vi "WLAN_SuperposedFrameBuild_MOD.vi"(4 "Modulation parameter LP":T1, 7 "Alpha":dbl min=0.0 max=1.0 step=0.05 format="%#_13g", 8 "error in (no error)":errorcluster, 9 "data in 2":i8[](array[numeric]) caption="input bit stream", 10 "Modulation parameter HP":T1, 11 "data in":i8[](array[numeric]) caption="input bit stream") -> (0 "error out":errorcluster, 2 "symbolsLP":cdb[](array[numeric]), 3 "symbolsHP":cdb[](array[numeric]))   [LabVIEW 2022 SP3]
panel:
  out "scrambled bits":i8[](array[numeric])
  out "size(s) 5":i32
  out "symbols":cdb[](array[numeric])
  out "output bit stream 4":i8[](array[numeric])
  out "output bit stream 3":i8[](array[numeric])
  out "subarray 2":i8[](array[numeric])
  out "subarray":i8[](array[numeric])
  out "size(s) 2":i32
  out "size(s) 6":i32
  out "size(s) 4":i32
  out "size(s) 3":i32
  out "size(s)":i32
  in  "data in 3":i8[](array[numeric]) caption="input bit stream"
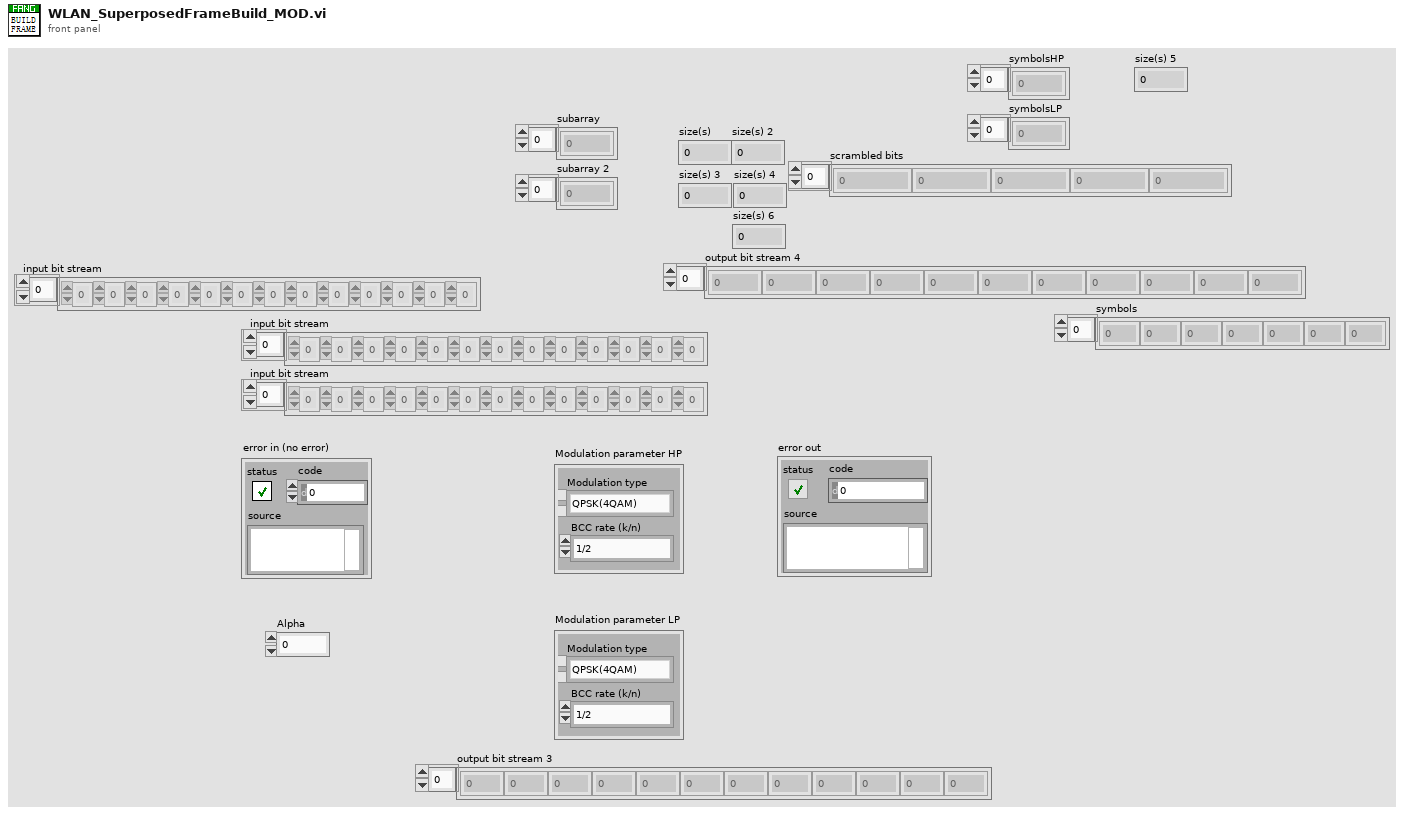
[diagram p1: front panel]
types:
  T1 = cluster{"Modulation type":enum16{"QPSK(4QAM)", "64QAM", "16QAM", "BPSK"}, "BCC rate (k/n)":enum16{"1/2", "2/3", "3/4"}}
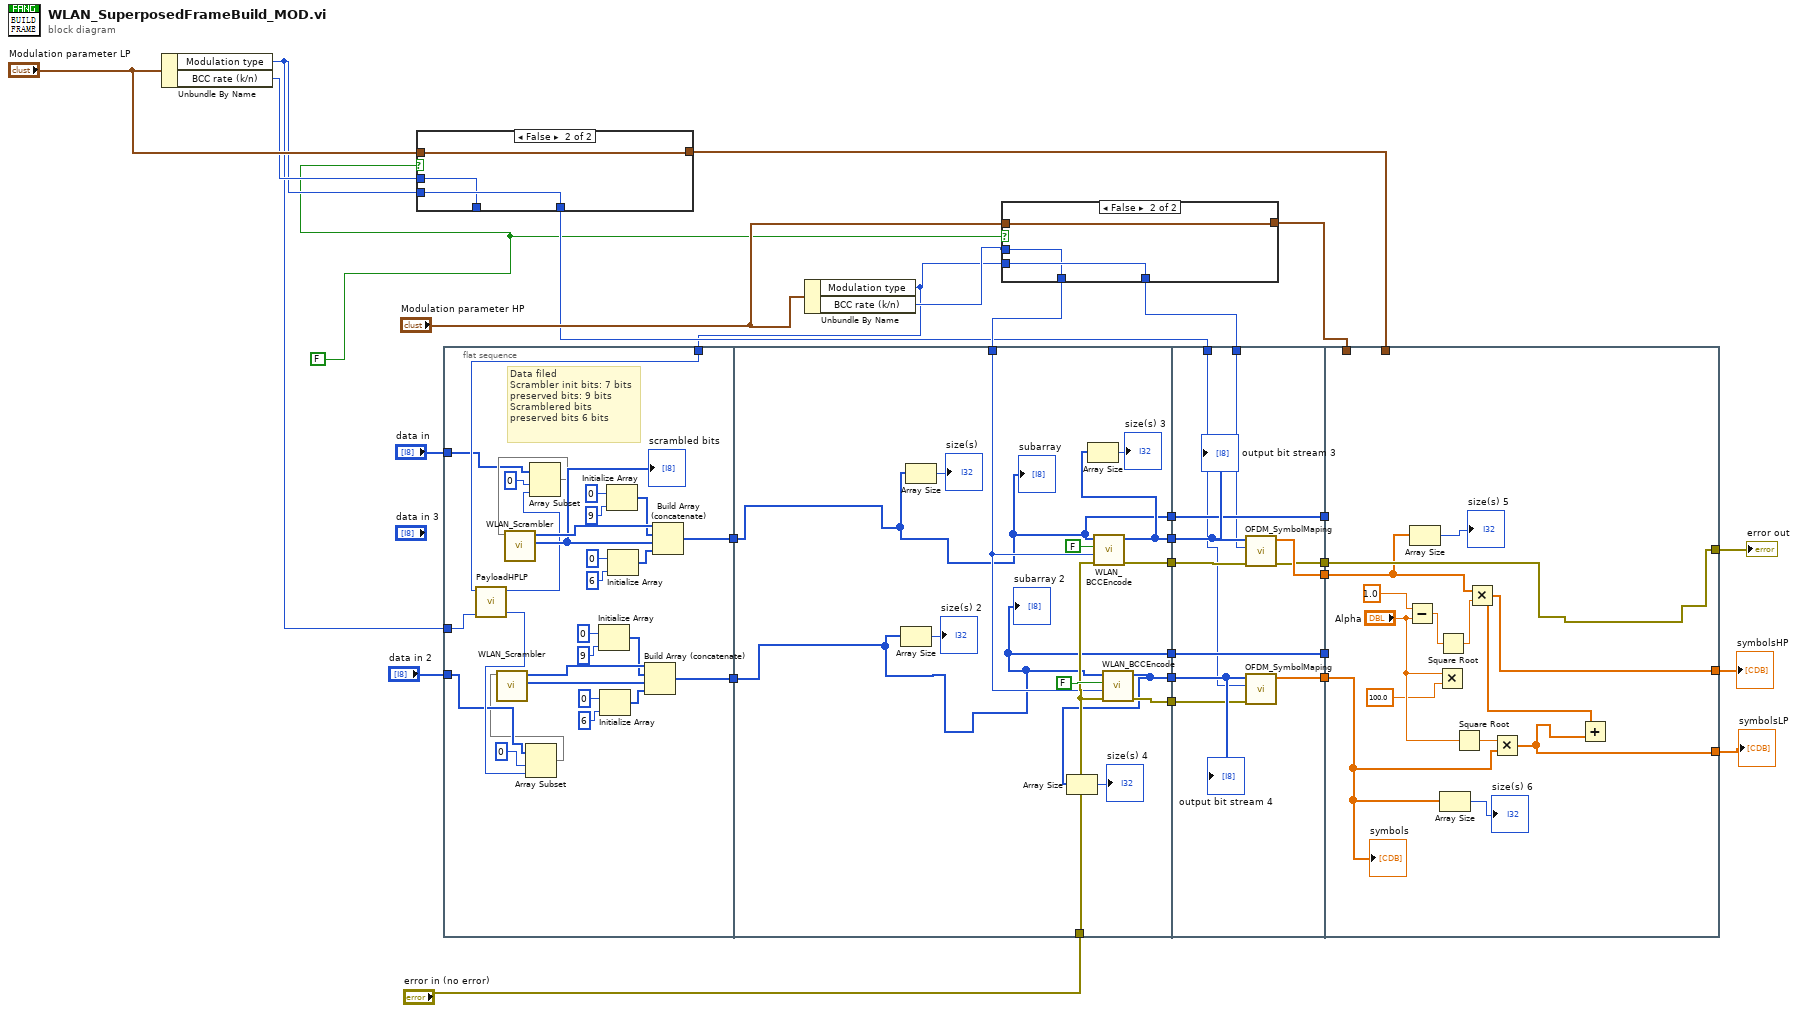
[diagram p0: block diagram]
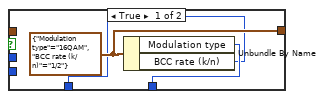
[diagram p2: hidden frame]
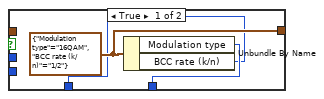
[diagram p3: hidden frame]
diagram:
  w1 = FALSE
  n1 = Unbundle By Name("Modulation parameter LP") -> ("Modulation type"=w5:enum16{"QPSK(4QAM)", "64QAM", "16QAM", "BPSK"}, "BCC rate (k/n)"=w8:enum16{"1/2", "2/3", "3/4"})
  n2 = case shown="False" w1 {
    tunnel: w5 -> [_ w37]
    tunnel: [w34 w37] -> w7
    tunnel: [w33 w36] -> w6
    tunnel: "Modulation parameter LP" -> [_ w36]
    tunnel: [w32 w35] -> _
    tunnel: w8 -> [_ w35]
    frame True {
      w33 = T1 {"Modulation type"=enum."16QAM", "BCC rate (k/n)"=enum."1/2"} ("Modulation parameter")
      n3 = Unbundle By Name(w33) -> ("Modulation type"=w34:enum16{"QPSK(4QAM)", "64QAM", "16QAM", "BPSK"}, "BCC rate (k/n)"=w32:enum16{"1/2", "2/3", "3/4"})
    }
    frame False {
    }
  }
  n4 = flat-sequence {
    tunnel: "data in" -> [w40]
    tunnel: [w57] -> w30
    tunnel: "data in 2" -> [w39]
    tunnel: [w48] -> w20
    tunnel: w5 -> [w47]
    tunnel: w4 -> [w46]
    tunnel: w30 -> [w67]
    tunnel: "error in (no error)" -> [w76]
    tunnel: [w78] -> w28
    tunnel: [w70] -> w27
    tunnel: w11 -> [w75]
    tunnel: [w67] -> w23
    tunnel: w20 -> [w66]
    tunnel: [w66] -> w19
    tunnel: [w69] -> w18
    tunnel: [w74] -> w16
    tunnel: w28 -> [w90]
    tunnel: w27 -> [w89]
    tunnel: w14 -> [w81]
    tunnel: [w88] -> w26
    tunnel: [w87] -> w25
    tunnel: w23 -> [w86]
    tunnel: [w86] -> w22
    tunnel: w19 -> [w84]
    tunnel: w18 -> [w85]
    tunnel: [w84] -> w17
    tunnel: w16 -> [w83]
    tunnel: [w82] -> w15
    tunnel: w7 -> [w80]
    tunnel: w13 -> [_]
    tunnel: w26 -> [w92]
    tunnel: w25 -> [w95]
    tunnel: [w95] -> w24
    tunnel: w22 -> [_]
    tunnel: w17 -> [_]
    tunnel: w15 -> [w99]
    tunnel: w6 -> [_]
    tunnel: [w94] -> w3
    tunnel: [w93] -> w2
    frame #0 {
      # "Data filed\nScrambler init bits: 7 bits\npreserved bits: 9 bits\nScramblered bits\npreserved bits 6 bits"
      n5 = call "PayloadHPLP.vi"("Modulation type LP"=w47, "Modulation type HP"=w46) -> ("Payload_LP"=w45:i32, "Payload_HP"=w42:i32)  [unwired: 8 in]
      n6 = Array Subset(array=w39, index=0, length=w45) -> (w38:i8[])
      n7 = call "WLAN_Scrambler.vi"("input bit stream"=w38) -> ("scrambled bits"=w52:i8[], "scrambler initial bit"=w56:i8[])  [unwired: 9 in]
      n8 = Array Subset(array=w40, index=0, length=w42) -> (w41:i8[])
      n9 = call "WLAN_Scrambler.vi"("input bit stream"=w41) -> ("scrambled bits"=w61:i8[], "scrambler initial bit"=w65:i8[])  [unwired: 9 in]
      "scrambled bits" <- w61
      n10 = Initialize Array(i8 0 ("element"), 9 ("dimension size")) -> (w55:i8[])
      n11 = Initialize Array(i8 0 ("element"), 6 ("dimension size")) -> (w49:i8[])
      n12 = Initialize Array(i8 0 ("element"), 9 ("dimension size")) -> (w64:i8[])
      n13 = Initialize Array(i8 0 ("element"), 6 ("dimension size")) -> (w58:i8[])
      n14 = Build Array (concatenate)(w56, w55, w52, w49) -> (w48:i8[])
      n15 = Build Array (concatenate)(w65, w64, w61, w58) -> (w57:i8[])
    }
    frame #1 {
      n16 = Array Size(array=w66) -> (size(s)=→"size(s) 2":i32)
      n17 = Array Size(array=w67) -> (size(s)=→"size(s)":i32)
      n18 = call "WLAN_BCCEncode.vi"("error in (no error)"=w76, "BCC rate (k/n)"=w75, "need add zeros?"=FALSE, "input bit stream"=w67) -> ("error out"=w78:errorcluster, "output bit stream 3"=w70:i8[])  [unwired: 6 in]
      n19 = Array Size(array=w70) -> (size(s)=→"size(s) 3":i32)
      n20 = call "WLAN_BCCEncode.vi"("error in (no error)"=w76, "BCC rate (k/n)"=w75, "need add zeros?"=FALSE, "input bit stream"=w66) -> ("error out"=w74:errorcluster, "output bit stream 3"=w69:i8[])  [unwired: 6 in]
      n21 = Array Size(array=w69) -> (size(s)=→"size(s) 4":i32)
      "subarray" <- w67
      "subarray 2" <- w66
    }
    frame #2 {
      n22 = call "OFDM_SymbolMaping.vi"("error in (no error)"=w90, "Modulation type"=w81, "input bit stream"=w89) -> ("error out"=w87:errorcluster, "symbols"=w88:cdb[])  [unwired: 7 in]
      n23 = call "OFDM_SymbolMaping.vi"("error in (no error)"=w83, "Modulation type"=w80, "input bit stream"=w85) -> ("symbols"=w82:cdb[])  [unwired: 7 in, 1 out]
      "output bit stream 3" <- w89
      "output bit stream 4" <- w85
    }
    frame #3 {
      n24 = Subtract(x=1.0, y="Alpha") -> (x-y=w101:dbl)
      n25 = Array Size(array=w92) -> (size(s)=→"size(s) 5":i32)
      n26 = Multiply(x="Alpha", y=100.0) -> ()  [unwired: 1 out]
      n27 = Square Root(x=w101) -> (sqrt(x)=w102:dbl)
      n28 = Array Size(array=w99) -> (size(s)=→"size(s) 6":i32)
      n29 = Square Root(x="Alpha") -> (sqrt(x)=w103:dbl)
      n30 = Multiply(x=w92, y=w102) -> (x*y=w94:cdb[])
      n31 = Multiply(x=w103, y=w99) -> (x*y=w93:cdb[])
      n32 = Add(x=w94, y=w93) -> ()  [unwired: 1 out]
      "symbols" <- w99
    }
  }
  n33 = Unbundle By Name("Modulation parameter HP") -> ("Modulation type"=w4:enum16{"QPSK(4QAM)", "64QAM", "16QAM", "BPSK"}, "BCC rate (k/n)"=w10:enum16{"1/2", "2/3", "3/4"})
  n34 = case shown="False" w1 {
    tunnel: w4 -> [_ w109]
    tunnel: [w106 w109] -> w14
    tunnel: [w105 w108] -> w13
    tunnel: "Modulation parameter HP" -> [_ w108]
    tunnel: [w104 w107] -> w11
    tunnel: w10 -> [_ w107]
    frame True {
      w105 = T1 {"Modulation type"=enum."16QAM", "BCC rate (k/n)"=enum."1/2"} ("Modulation parameter")
      n35 = Unbundle By Name(w105) -> ("Modulation type"=w106:enum16{"QPSK(4QAM)", "64QAM", "16QAM", "BPSK"}, "BCC rate (k/n)"=w104:enum16{"1/2", "2/3", "3/4"})
    }
    frame False {
    }
  }
  "error out" <- w24
  "symbolsHP" <- w3
  "symbolsLP" <- w2
